vi "Read IRuleFileParser.vi"(10 "Path":path, 11 "CDependencyInspection in":refnum<class "CDependencyInspection.lvclass">) -> (0 "error out":errorcluster, 1 "IRuleFileParser":refnum<class "IRuleFileParser.lvclass">, 3 "CDependencyInspection out":refnum<class "CDependencyInspection.lvclass">)   [LabVIEW 2020, in "DependencyInspection.lvlib" / "CDependencyInspection.lvclass"]
uses:
  CDependencyInspection.lvclass
  ExtensionInterfaces/IRuleFileParser/IRuleFileParser.lvclass
  CDependencyInspection.lvclass/CDependencyInspection.ctl
  d930f320-e5c5-426c-99f6-64d57fd880dc.vi
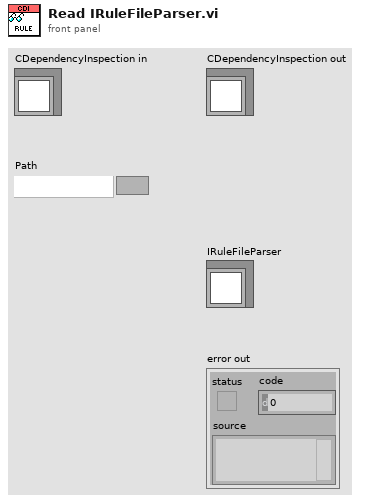
[diagram p1: front panel]
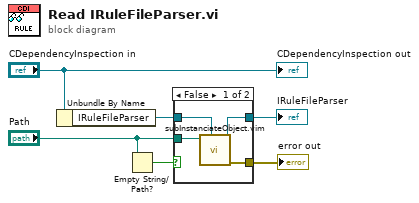
[diagram p0: block diagram]
diagram:
  n1 = Unbundle By Name("CDependencyInspection in") -> ("IRuleFileParser"=w4:refnum<class "IRuleFileParser.lvclass">)
  n2 = Empty String/Path?(string/path="Path") -> (empty?=w3:bool)
  n3 = case shown="False" w3 {
    tunnel: "Path" -> [w10 _]
    tunnel: w4 -> [w9 w11]
    tunnel: [w8 w11] -> w2
    tunnel: [w7 _] -> w1
    frame False {
      n4 = call "subInstanciateObject.vim"("Target object"=w9, "Class path"=w10) -> ("error out"=w7:errorcluster, "Object"=w8:refnum<class "IRuleFileParser.lvclass">)  [unwired: 8 in]
    }
    frame True {
    }
  }
  "IRuleFileParser" <- w2
  "error out" <- w1
  "CDependencyInspection out" <- "CDependencyInspection in"
